vi "Check Duplicate Node_IDs.vi"(8 "errors in":refnum<class "MultiErrors.lvclass">, 11 "ID Name Map":map{i32, string[]}(c390)) -> (0 "errors out":refnum<class "MultiErrors.lvclass">)   [LabVIEW 2025, in "VolatusConfig.lvlib"]
uses:
  VolatusConfig.lvlib
  VolatusErrorUtilities/MultiErrors/MultiErrors.lvclass
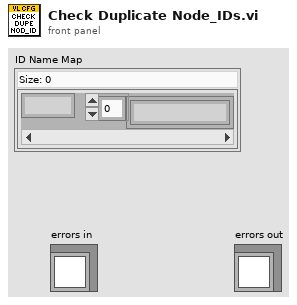
[diagram p1: front panel]
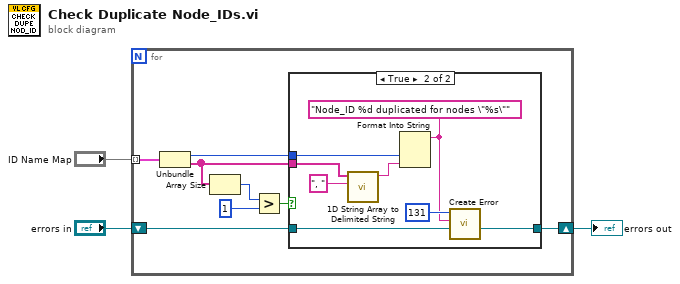
[diagram p0: block diagram]
diagram:
  n1 = for {
    shift-right: [w10] -> w2
    shift-left: "errors in" -> [w11]
    tunnel: "ID Name Map" -> [w9] mode=indexing
    n2 = Unbundle(w9) -> ("ID"=w5:i32, "Nodes"=w4:string[])
    n3 = Array Size(array=w4) -> (size(s)=w8:i32)
    n4 = Greater?(x=w8, y=1) -> (0:w6:bool)
    n5 = case shown="True" w6 {
      tunnel: w11 -> [w12 w16]
      tunnel: [w12 w15] -> w10
      tunnel: w5 -> [_ w18]
      tunnel: w4 -> [_ w20]
      frame False {
      }
      frame True {
        w13 = "Node_ID %d duplicated for nodes \"%s\"" ("format string")
        n6 = call <vilib>:"1D String Array to Delimited String.vi"("delimiter"=", ", "string array"=w20) -> ("delimited string"=w17:string)  [unwired: 9 in]
        n7 = Format Into String(format string=w13, w18, w17) -> ()  [unwired: 2 in, 2 out]
        n8 = call "Create Error.vi"("MultiErrors in"=w16, "Message"=w13, "Code"=131) -> ("MultiErrors out"=w15:refnum<class "MultiErrors.lvclass">)  [unwired: 8 in]
      }
    }
  }
  "errors out" <- w2
